vi "Error Handler.vi"(8 "error in (no error)":errorcluster, 11 "Modbus in":refnum<class "Modbus.lvclass">) -> (0 "error out":errorcluster, 3 "Modbus out":refnum<class "Modbus.lvclass">)   [LabVIEW 2026, in "Modbus.lvlib" / "Modbus.lvclass"]
uses:
  Modbus.lvclass
  Modbus.lvclass/Modbus.ctl
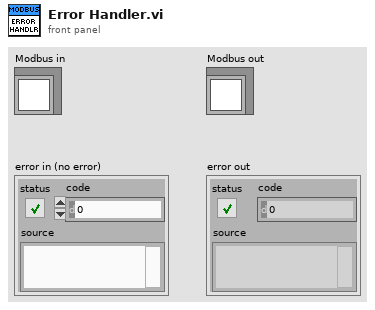
[diagram p1: front panel]
types:
  T1 = map{i32, cluster{"Status":bool, "Message":string}}
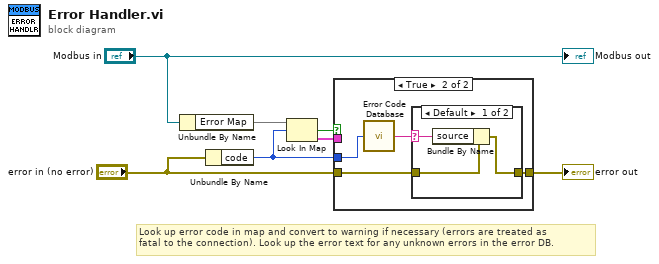
[diagram p0: block diagram]
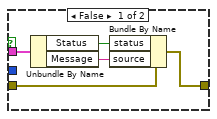
[diagram p2: hidden frame]
diagram:
  # "Look up error code in map and convert to warning if necessary (errors are treated as\nfatal to the connection). Look up the error text for any unknown errors in the error DB."
  n1 = Unbundle By Name("Modbus in") -> ("Error Map"=w2:T1)
  n2 = Unbundle By Name("error in (no error)") -> ("code"=w1:i32)
  n3 = Look In Map(map=w2, key=w1) -> (key not found?=w4:bool, value=w3:cluster{"Status":bool, "Message":string})  [unwired: 1 in]
  n4 = case shown="True" w4 {
    tunnel: "error in (no error)" -> [w12 w15]
    tunnel: [w11 w14] -> w6
    tunnel: w3 -> [w10 _]
    tunnel: w1 -> [_ w13]
    frame False {
      n5 = Unbundle By Name(w10) -> ("Status"=w9:bool, "Message"=w8:string)
      n6 = Bundle By Name(cluster=w12, "status"=w9, "source"=w8) -> (w11:errorcluster)
    }
    frame True {
      n7 = call <vilib>:"Error Code Database.vi"("Error Code"=w13) -> ("Error Text"=w16:string)
      n8 = case shown="Default" w16 {
        selector: w16 -> [w18 _]
        tunnel: w15 -> [w19 w20]
        tunnel: [w17 w20] -> w14
        frame Default {
          n9 = Bundle By Name(cluster=w19, "source"=w18) -> (w17:errorcluster)
        }
        frame "" {
        }
      }
    }
  }
  "error out" <- w6
  "Modbus out" <- "Modbus in"
